vi "Connect to PS3 Controller.vi"(7 "error in (no error)":errorcluster) -> (0 "error out":errorcluster, 2 "device ID 2":refnum<k1>)   [LabVIEW 2014]
panel:
  out "ID":i32
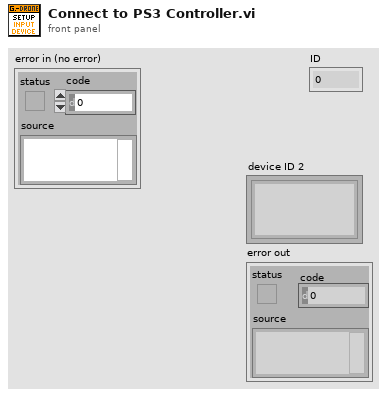
[diagram p1: front panel]
types:
  T1 = cluster{"axes total":u32, "buttons total":u32, "pov total":u32, "device name":string}[]
  T2 = cluster{"axes total":u32, "buttons total":u32, "pov total":u32, "device name":string}
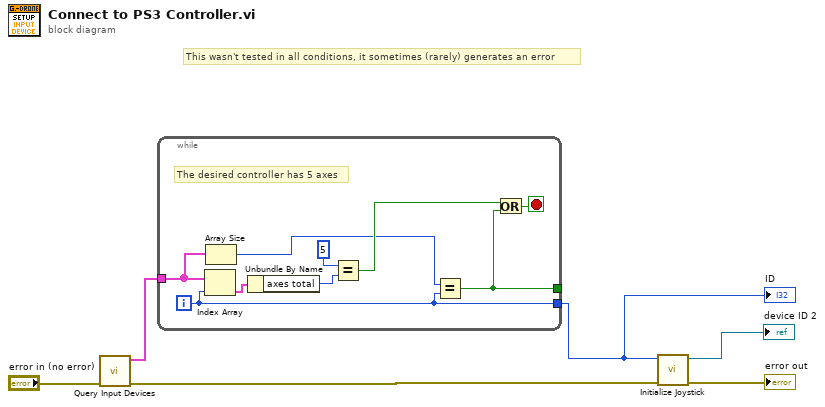
[diagram p0: block diagram]
diagram:
  # "This wasn't tested in all conditions, it sometimes (rarely) generates an error"
  n1 = call <vilib>:"Query Input Devices.vi"("error in (no error)"="error in (no error)") -> ("error out"=w4:errorcluster, "joystick info"=w6:T1)  [unwired: 7 in, 2 out]
  n2 = while {
    tunnel: w6 -> [w9]
    tunnel: [w10] -> w2
    tunnel: [w8] -> _
    i -> [w10]
    stop <- w12 stop-if-true
    # "The desired controller has 5 axes"
    n3 = Index Array(array=w9, index=w10) -> (element=w15:T2)
    n4 = Array Size(array=w9) -> (size(s)=w7:i32)
    n5 = Unbundle By Name(w15) -> ("axes total"=w13:u32)
    n6 = Equal?(x=u32 5 ("y"), y=w13) -> (x = y?=w11:bool)
    n7 = Equal?(x=w7, y=w10) -> (x = y?=w8:bool)
    n8 = Or(x=w11, y=w8) -> (x .or. y?=w12:bool)
  }
  "ID" <- w2
  n9 = call <vilib>:"Initialize Joystick.vi"("error in (no error)"=w4, "device index"=w2) -> ("error out"=→"error out":errorcluster, "device ID"=→"device ID 2":refnum<k1>)  [unwired: 8 in]
